vi "From CSV File.vi"(8 "error in (no error)":errorcluster, 9 "Path":path, 10 "engine in":refnum<class "engine configuration.lvclass">, 11 "PID Module editor node in":refnum<class "PID Module editor node.lvclass">) -> (0 "error out":errorcluster, 1 "Update":bool, 2 "engine out":refnum<class "engine configuration.lvclass">, 3 "PID Module editor node out":refnum<class "PID Module editor node.lvclass">)   [LabVIEW 2015, in "PID Module editor node.lvclass"]
uses:
  PID Module editor node.lvclass
  <vilib>/NI/Module Execution Interface/Engine Configuration/engine configuration.lvclass
  module/configuration/PID Module configuration.lvclass
  <vilib>/NI/Configuration Framework/serializable configuration/NISE_CEF_serializable configuration.lvclass/NISE_CEF_serializable configuration.ctl
  module/configuration/PID Module configuration.lvclass/PID Module configuration.ctl
  <vilib>/Utility/LVClass/Get LV Class Name.vi
  <vilib>/NI/Configuration Framework/error generator/NISE_error generator.vi
  <vilib>/NI/Tag Bus Module Framework/channel/TBM channel.lvclass
  <vilib>/NI/Configuration Framework/serializable configuration/NISE_CEF_serializable configuration.lvclass
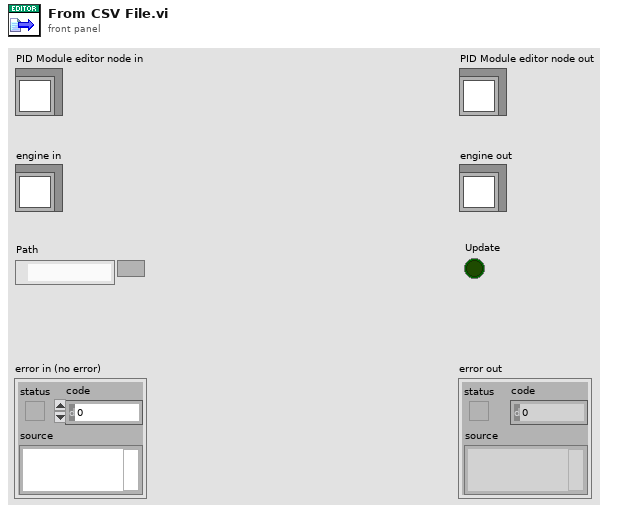
[diagram p1: front panel]
types:
  T1 = typedef "PID Module configuration.lvclass/Line.ctl" = cluster{"PID ID":string, "Setpoint":refnum<class "TBM channel.lvclass">, "Variable":refnum<class "TBM channel.lvclass">, "Output":refnum<class "TBM channel.lvclass">, "Output High":refnum<class "TBM channel.lvclass">, "Output Low":refnum<class "TBM channel.lvclass">, "P":refnum<class "TBM channel.lvclass">, "I":refnum<class "TBM channel.lvclass">, "D":refnum<class "TBM channel.lvclass">}
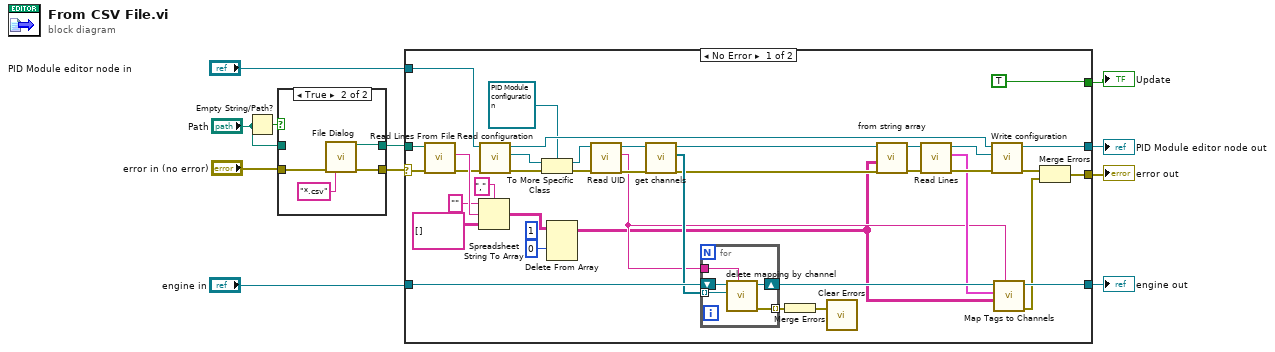
[diagram p0: block diagram]
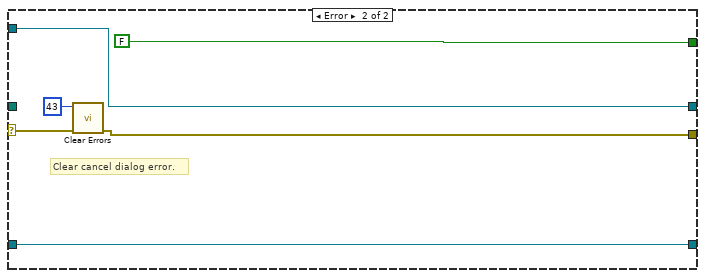
[diagram p2: hidden frame]
diagram:
  n1 = Empty String/Path?(string/path="Path") -> (empty?=w11:bool)
  n2 = case shown="True" w11 {
    tunnel: "error in (no error)" -> [w12 w16]
    tunnel: [w12 w15] -> w7
    tunnel: [w13 w14] -> w8
    tunnel: "Path" -> [w13 _]
    frame False {
    }
    frame True {
      n3 = call "File Dialog"("error in"=w16, "pattern (all files)"="*.csv") -> ("selected path"=w14:path, "error out"=w15:errorcluster)  [unwired: 10 in, 2 out]
    }
  }
  n4 = case shown="No Error" w7 {
    selector: w7 -> [w49 w64]
    tunnel: [w39 w63] -> w1
    tunnel: [w33 w66] -> w3
    tunnel: "PID Module editor node in" -> [w38 w66]
    tunnel: w8 -> [w54 _]
    tunnel: [TRUE ("Update") FALSE ("Update")] -> w4
    tunnel: "engine in" -> [w46 w61]
    tunnel: [w40 w61] -> w2
    frame No Error {
      n5 = call <vilib>:"Read Lines From File.vi"("file path (dialog if empty)"=w54, "error in (not an error)"=w49) -> ("line string"=w52:string, "error out"=w37:errorcluster)  [unwired: 5 in, 1 out]
      n6 = Spreadsheet String To Array(delimiter (Tab)=",", format string="", spreadsheet string=w52, array type (2D Dbl)=string[][] [] ("type (empty)")) -> (array=w21:string[][])
      n7 = call-dynamic "Read configuration.vi"("error in"=w37, "PID Module editor node in"=w38) -> ("error out"=w35:errorcluster, "configuration"=w36:refnum<class "NISE_CEF_serializable configuration.lvclass">, "PID Module editor node out"=w34:refnum<class "PID Module editor node.lvclass">)  [unwired: 7 in]
      n8 = To More Specific Class(target class=refnum<class "PID Module configuration.lvclass"> refnum ("tag bus configurable plugin module configuration"), reference=w36, error in=w35) -> (specific class reference=w48:refnum<class "PID Module configuration.lvclass">, error out=w42:errorcluster)
      n9 = Delete From Array(array=w21, length=1, index (row)=0) -> (array with subset deleted=w20:string[][])  [unwired: 1 in, 1 out]
      n10 = call <vilib>:"Read UID.vi"("error in"=w42, "configuration in"=w48) -> ("error out"=w30:errorcluster, "instance id"=w22:string, "configuration out"=w47:refnum<class "PID Module configuration.lvclass">)  [unwired: 7 in]
      n11 = call-dynamic "get channels.vi"("PID Module configuration in"=w47) -> ("channels"=w45:refnum<class "TBM channel.lvclass">[], "PID Module configuration out"=w43:refnum<class "PID Module configuration.lvclass">)  [unwired: 9 in]
      n12 = for {
        tunnel: w22 -> [w59]
        tunnel: w45 -> [w58] mode=indexing
        tunnel: [w57] -> w44 mode=indexing
        shift-right: [w56] -> w41
        shift-left: w46 -> [w60]
        n13 = call <vilib>:"delete mapping by channel.vi"("owner ID"=w59, "channel"=w58, "engine configuration in"=w60) -> ("error out"=w57:errorcluster, "engine configuration out"=w56:refnum<class "engine configuration.lvclass">)  [unwired: 7 in]
      }
      n14 = Merge Errors(w44) -> (w31:errorcluster)
      n15 = call <vilib>:"Clear Errors.vi"("error in (no error)"=w31) -> ()  [unwired: 5 in, 2 out]
      n16 = call-dynamic "from string array.vi"("error in (no error)"=w30, "String Array"=w20, "PID Module configuration in"=w43) -> ("error out"=w28:errorcluster, "PID Module configuration out"=w25:refnum<class "PID Module configuration.lvclass">)  [unwired: 7 in]
      n17 = call "Read Lines.vi"("error in (no error)"=w28, "PID Module configuration in"=w25) -> ("error out"=w27:errorcluster, "Lines"=w23:T1[], "PID Module configuration out"=w26:refnum<class "PID Module configuration.lvclass">)  [unwired: 7 in]
      n18 = call-dynamic "Write configuration.vi"("error in"=w27, "configuration"=w26, "PID Module editor node in"=w34) -> ("error out"=w32:errorcluster, "PID Module editor node out"=w33:refnum<class "PID Module editor node.lvclass">)  [unwired: 7 in]
      n19 = call "Map Tags to Channels.vi"("instance id"=w22, "String Array"=w20, "Lines"=w23, "engine configuration in"=w41) -> ("error out"=w24:errorcluster, "engine configuration out"=w40:refnum<class "engine configuration.lvclass">)  [unwired: 6 in]
      n20 = Merge Errors(w32, w24) -> (w39:errorcluster)
    }
    frame Error {
      # "Clear cancel dialog error."
      n21 = call <vilib>:"Clear Errors.vi"("error in (no error)"=w64, "specific error code to clear (0: all)"=43) -> ("error out"=w63:errorcluster)  [unwired: 4 in, 1 out]
    }
  }
  "error out" <- w1
  "PID Module editor node out" <- w3
  "Update" <- w4
  "engine out" <- w2
